vi "SetFrequency.vi"(8 "error in (no error)":errorcluster, 10 "Freq":sgl[](array[numeric]), 11 "M5Stack I2C 8Ch Servo in":refnum<class "M5Stack I2C 8Ch Servo.lvclass">) -> (0 "error out":errorcluster, 3 "M5Stack I2C 8Ch Servo out":refnum<class "M5Stack I2C 8Ch Servo.lvclass">)   [LabVIEW 2020, in "CTI-Peripheral.lvlib" / "M5Stack I2C 8Ch Servo.lvclass"]
uses:
  M5Stack I2C 8Ch Servo.lvclass
  M5Stack I2C 8Ch Servo.lvclass/M5Stack I2C 8Ch Servo.ctl
  Private/registers.ctl
  CTI/I2C Connection/I2C Connection.lvclass/I2C Connection.ctl
  CTI/Session/I2C Write Data.vi
  CTI/I2C Connection/I2C Connection.lvclass
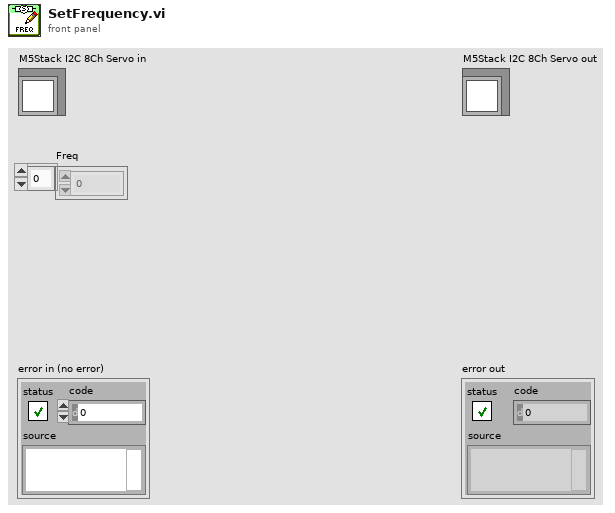
[diagram p1: front panel]
types:
  T1 = typedef "CTI-Peripheral.lvlib/M5Stack I2C 8Ch Servo.lvclass/registers.ctl" = u8
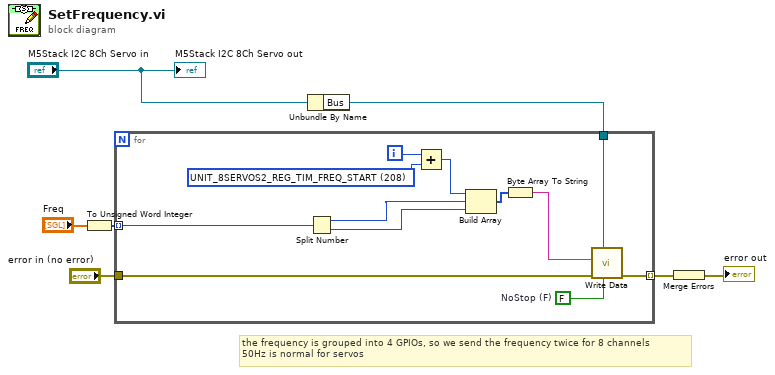
[diagram p0: block diagram]
diagram:
  # "the frequency is grouped into 4 GPIOs, so we send the frequency twice for 8 channels\n50Hz is normal for servos"
  n1 = To Unsigned Word Integer(number="Freq") -> (unsigned 16bit integer=w6:u16[])
  n2 = Unbundle By Name("M5Stack I2C 8Ch Servo in") -> ("Bus"=w7:refnum<class "I2C Connection.lvclass">)
  n3 = for {
    tunnel: w7 -> [w16]
    tunnel: w6 -> [w9] mode=indexing
    tunnel: "error in (no error)" -> [w12]
    tunnel: [w13] -> w2 mode=indexing
    i -> [w8]
    w15 = T1 208 items=["UNIT_8SERVOS2_REG_MODE_START"=0, "UNIT_8SERVOS2_REG_INPUT_PULL_START"=16, "UNIT_8SERVOS2_REG_INPUT_STATUS_START"=32, "UNIT_8SERVOS2_REG_OUTPUT_STATUS_START"=48, "UNIT_8SERVOS2_REG_ADC_START"=64, "UNIT_8SERVOS2_REG_SERVO_START"=80, "UNIT_8SERVOS2_REG_RGB_CONF_START"=96, "UNIT_8SERVOS2_REG_PWM_DUTY_START"=112, "UNIT_8SERVOS2_REG_RGB_BUFFER_START"=128, "UNIT_8SERVOS2_REG_TIM_FREQ_START"=208, "UNIT_8SERVOS2_REG_UID_START"=224, "UNIT_8SERVOS2_REG_UID_END"=235, "UNIT_8SERVOS2_REG_SYS_ANALOG_START"=240, "UNIT_8SERVOS2_REG_ADDR_OFFSET"=248, "UNIT_8SERVOS2_REG_I2C_ADDR_REFRESH"=252, "UNIT_8SERVOS2_REG_VERSION"=254, "UNIT_8SERVOS2_REG_I2C_ADDR"=255] ("Registers")
    w19 = FALSE  # NoStop (F)
    n4 = Split Number(x=w9) -> (hi(x)=w11:u8, lo(x)=w10:u8)
    n5 = Add(x=w8, y=w15) -> (x+y=w14:i32)
    n6 = Build Array(w14, w11, w10) -> (w18:i32[])
    n7 = Byte Array To String(unsigned byte array=w18) -> (string=w17:string)
    n8 = call "Write Data.vi"("NoStop (F)"=w19, "I2C Connection"=w16, "error in (no error)"=w12, "Data"=w17) -> ("error out"=w13:errorcluster)  [unwired: 7 in]
  }
  n9 = Merge Errors(w2) -> (→"error out":errorcluster)
  "M5Stack I2C 8Ch Servo out" <- "M5Stack I2C 8Ch Servo in"
